vi "delete directory from protected Windows location.vi"(8 "error in":errorcluster, 11 "directory":path=path "C:/Program Files (x86)/National Instruments/RT Images/User Components/C Series Module Detection") -> (0 "error out":errorcluster, 2 "deleted?":bool)   [LabVIEW 2014]
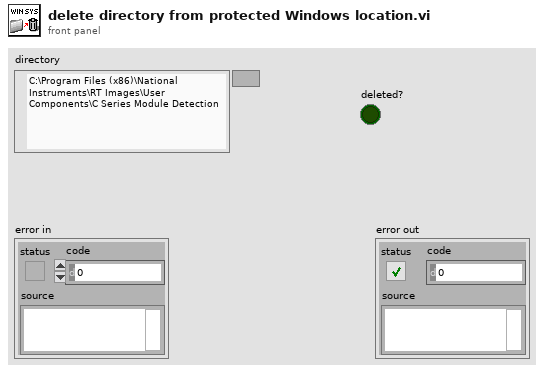
[diagram p1: front panel]
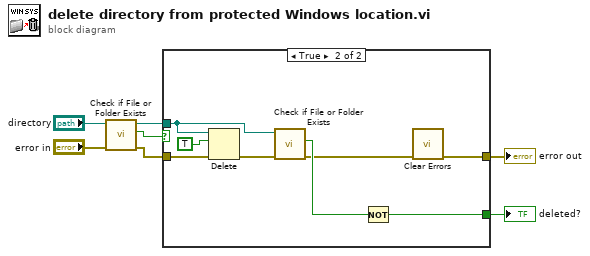
[diagram p0: block diagram]
diagram:
  n1 = call <vilib>:"Check if File or Folder Exists.vi"("error in (no error)"="error in", "path"="directory") -> ("error out"=w3:errorcluster, "file or folder exists?"=w4:bool, "dup path"=w5:path)  [unwired: 7 in]
  n2 = case shown="True" w4 {
    tunnel: [w8 w9] -> w2
    tunnel: [_ w15] -> w7
    tunnel: w5 -> [_ w11]
    tunnel: w3 -> [w8 w14]
    frame False {
    }
    frame True {
      n3 = Delete(path (use dialog)=w11, entire hierarchy (F)=TRUE ("overwrite (F)"), error in=w14) -> (error out=w12:errorcluster)  [unwired: 2 in, 2 out]
      n4 = call <vilib>:"Check if File or Folder Exists.vi"("error in (no error)"=w12, "path"=w11) -> ("error out"=w10:errorcluster, "file or folder exists?"=w13:bool)  [unwired: 7 in, 1 out]
      n5 = Not(x=w13) -> (.not. x?=w15:bool)
      n6 = call <vilib>:"Clear Errors.vi"("error in (no error)"=w10) -> ("error out"=w9:errorcluster)  [unwired: 5 in, 1 out]
    }
  }
  "error out" <- w2
  "deleted?" <- w7
